vi "relay-sample.vi"() -> ()   [LabVIEW 2020]
uses:
  <vilib>/Rock Robotics/SystemInterfaces/DIO/FPGA_DIORelayChannel.ctl
  <vilib>/Rock Robotics/WPI/Relay/WPI_RelayDirection.ctl
  <vilib>/Rock Robotics/WPI/Relay/WPI_RelayValue.ctl
panel:
  in  "RELAY\nREVERSE":bool
  in  "RELAY\nFORWARD":bool
  in  "RELAY\nCONTROL":bool
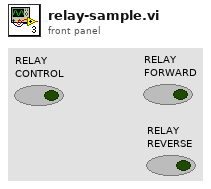
[diagram p1: front panel]
types:
  T1 = typedef "WPI_RelayValue.ctl" = enum16{"Off", "On", "Forward", "Reverse"}
  T2 = typedef "WPI_RelayDirection.ctl" = enum16{"Both directions", "Forward only", "Reverse only"}
  T3 = typedef "FPGA_DIORelayChannel.ctl" = enum8{"Relay 0", "Relay 1", "Relay 2", "Relay 3", "Invalid"}
  T4 = typedef "WPI_RelayDevRef.ctl" = cluster{"DevStatus":errorcluster, "Relay Channel":T3, "Relay Direction":T2}
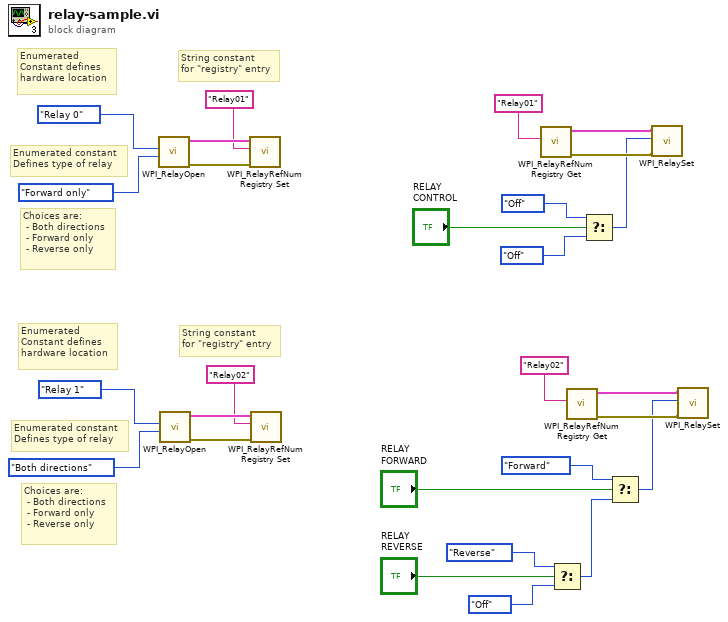
[diagram p0: block diagram]
diagram:
  # "Choices are:\n - Both directions\n - Forward only\n - Reverse only"
  # "String constant\nfor \"registry\" entry"
  # "Enumerated constant\nDefines type of relay"
  # "Enumerated\nConstant defines\nhardware location"
  # "Choices are:\n - Both directions\n - Forward only\n - Reverse only"
  # "String constant\nfor \"registry\" entry"
  # "Enumerated constant\nDefines type of relay"
  # "Enumerated\nConstant defines\nhardware location"
  n1 = call <vilib>:"WPI_RelayOpen.vi"("Relay Direction"=WPI_RelayDirection."Forward only", "Relay Channel"=FPGA_DIORelayChannel."Relay 0") -> ("error out"=w23:errorcluster, "RelayDevRef"=w27:T4)  [unwired: 8 in]
  n2 = call <vilib>:"WPI_RelayOpen.vi"("Relay Direction"=WPI_RelayDirection."Both directions", "Relay Channel"=FPGA_DIORelayChannel."Relay 1") -> ("error out"=w18:errorcluster, "RelayDevRef"=w22:T4)  [unwired: 8 in]
  n3 = call <vilib>:"WPI_RelayRefNum Registry Set.vi"("error in (no error)"=w23, "refnum name"="Relay01", "RelayDevRef"=w27) -> ()  [unwired: 7 in, 2 out]
  n4 = call <vilib>:"WPI_RelayRefNum Registry Set.vi"("error in (no error)"=w18, "refnum name"="Relay02", "RelayDevRef"=w22) -> ()  [unwired: 7 in, 2 out]
  n5 = call <vilib>:"WPI_RelayRefNum Registry Get.vi"("refnum name"="Relay01") -> ("error out"=w16:errorcluster, "RelayDevRef"=w17:T4)  [unwired: 9 in]
  n6 = Select(t=WPI_RelayValue."Reverse" ("RelayValue"), s="RELAY\nREVERSE", f=WPI_RelayValue."Off" ("RelayValue")) -> (s? t:f=w1:T1)
  n7 = call <vilib>:"WPI_RelayRefNum Registry Get.vi"("refnum name"="Relay02") -> ("error out"=w9:errorcluster, "RelayDevRef"=w10:T4)  [unwired: 9 in]
  n8 = Select(t=WPI_RelayValue."Off" ("RelayValue"), s="RELAY\nCONTROL", f=WPI_RelayValue."Off" ("RelayValue")) -> (s? t:f=w12:T1)
  n9 = Select(t=WPI_RelayValue."Forward" ("RelayValue"), s="RELAY\nFORWARD", f=w1) -> (s? t:f=w6:T1)
  n10 = call <vilib>:"WPI_RelaySet.vi"("error in (no error)"=w16, "RelayValue"=w12, "RelayDevRef"=w17) -> ()  [unwired: 7 in, 2 out]
  n11 = call <vilib>:"WPI_RelaySet.vi"("error in (no error)"=w9, "RelayValue"=w6, "RelayDevRef"=w10) -> ()  [unwired: 7 in, 2 out]
